vi "MTD.vi"(0 "MTD Input":cdb[](array[numeric]), 1 "NFFT":i32, 2 "NPRI":i32, 3 "PRF":i32) -> (7 "MTD Output":cdb[](array[numeric]), 9 "MTD_Max":cdb[](array[numeric]), 10 "Max_Index":dbl[](array[numeric]))   [LabVIEW 2012]
uses:
  <vilib>/Analysis/2dsp.llb/Complex FFT.vi
  <vilib>/Analysis/NI_AALPro.lvlib
panel:
  out "Input Size":i32
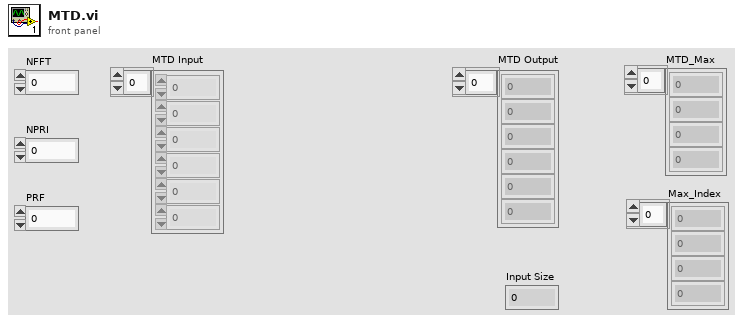
[diagram p1: front panel]
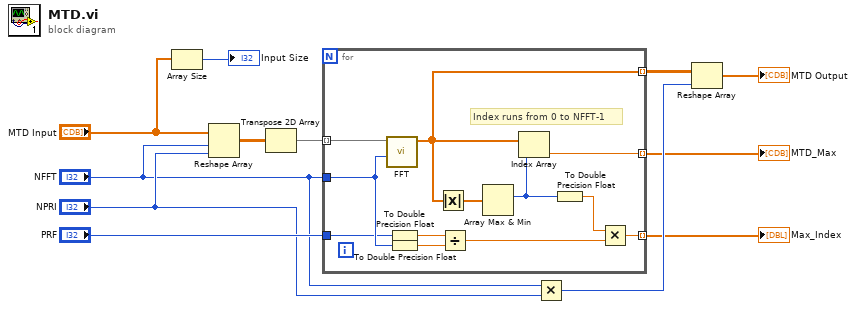
[diagram p0: block diagram]
diagram:
  n1 = Array Size(array="MTD Input") -> (size(s)=→"Input Size":i32)
  n2 = Reshape Array("MTD Input", "NFFT", "NPRI") -> (w4:cdb[][])
  n3 = Transpose 2D Array(2D array=w4) -> (transposed array=w10:cdb[][])
  n4 = for {
    tunnel: "NFFT" -> [w23]
    tunnel: [w15] -> w9 mode=indexing
    tunnel: [w13] -> w6 mode=indexing
    tunnel: [w17] -> w5 mode=indexing
    tunnel: "PRF" -> [w20]
    tunnel: w10 -> [w16] mode=indexing
    # "Index runs from 0 to NFFT-1"
    n5 = call-poly <vilib>:"FFT.vi"("FFT size"=w23, "X"=w16) -> ("FFT {X}"=w15:cdb[])  [unwired: 8 in, 1 out]
    n6 = To Double Precision Float(number=w20) -> (double precision float=w21:dbl)
    n7 = To Double Precision Float(number=w23) -> (double precision float=w22:dbl)
    n8 = Absolute Value(x=w15) -> (abs(x)=w24:dbl[])
    n9 = Divide(x=w21, y=w22) -> (x/y=w19:dbl)
    n10 = Array Max & Min(array=w24) -> (max index (indices)=w14:i32)  [unwired: 3 out]
    n11 = Index Array(array=w15, index=w14) -> (element=w13:cdb)
    n12 = To Double Precision Float(number=w14) -> (double precision float=w18:dbl)
    n13 = Multiply(x=w18, y=w19) -> (x*y=w17:dbl)
  }
  "MTD_Max" <- w6
  "Max_Index" <- w5
  n14 = Multiply(x="NFFT", y="NPRI") -> (x*y=w8:i32)
  n15 = Reshape Array(w9, w8) -> (→"MTD Output":cdb[])
